vi "set Marker Table OnOff.vi"(8 "error in (no error)":errorcluster, 10 "Marker Table On?":bool, 11 "FSV-40N in":refnum<class "FSV-40N.lvclass">) -> (0 "error out":errorcluster, 3 "FSV-40N out":refnum<class "FSV-40N.lvclass">)   [LabVIEW 2023, in "Spectrum Analyzer.lvlib" / "FSV-40N.lvclass"]
uses:
  FSV-40N.lvclass
  FSV-40N.lvclass/FSV-40N.ctl
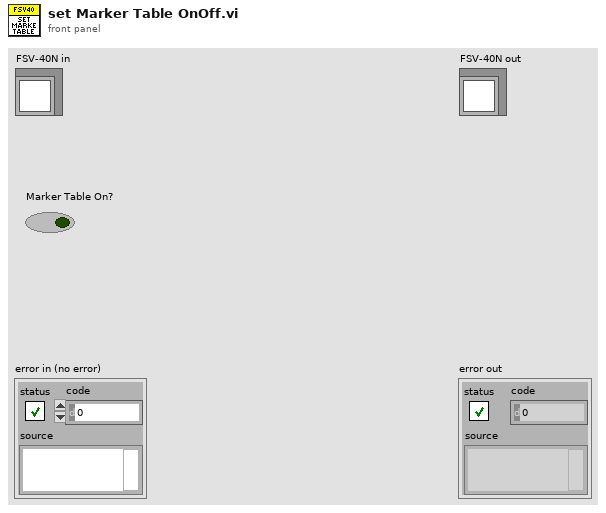
[diagram p1: front panel]
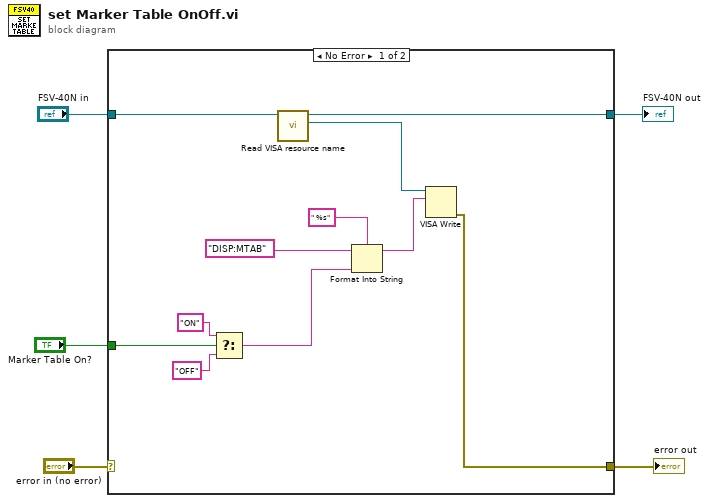
[diagram p0: block diagram]
diagram:
  n1 = case shown="No Error" "error in (no error)" {
    selector: "error in (no error)" -> [_ w17]
    tunnel: "FSV-40N in" -> [w16 w18]
    tunnel: [w11 w18] -> w4
    tunnel: [w13 w17] -> w2
    tunnel: "Marker Table On?" -> [w9 _]
    frame No Error {
      n2 = Select(t="ON" ("initial string"), s=w9, f="OFF" ("initial string")) -> (s? t:f=w6:string)
      n3 = call "Read VISA resource name.vi"("FSV-40N in"=w16) -> ("VISA resource name"=w12:refnum<visa-resource-name>, "FSV-40N out"=w11:refnum<class "FSV-40N.lvclass">)  [unwired: 8 in, 1 out]
      n4 = Format Into String(format string=" %s", initial string="DISP:MTAB", w6) -> (resulting string=w14:string)  [unwired: 1 in, 1 out]
      n5 = VISA Write(VISA resource name=w12, write buffer=w14) -> (error out=w13:errorcluster)  [unwired: 1 in, 2 out]
    }
    frame Error {
    }
  }
  "error out" <- w2
  "FSV-40N out" <- w4
